vi "DiffDriveTrainSim_ClampInput.vi"(9 "BatteryVoltage":dbl, 11 "U":T1) -> (0 "Size Coerced":bool, 3 "Normalized U":T1)   [LabVIEW 2019, in "Trajectory_Library.lvlib"]
doc: "Clamp the input vector such that no element exceeds the battery voltage. If any does, the relative magnitudes of the input will be maintained.\n \nInputs:\n - u -- The input vector.\n - BatteryVoltage -- The battery voltage (volts)\n\nOutputs:\n - NormalizedU -- The normalized input.\n - SizeCoerced -- If TRUE, an error occured."
uses:
  Trajectory_Library.lvlib
  <vilib>/Analysis/Matrix/Datatypes/RealMatrix.ctl
  <vilib>/Analysis/Matrix/NI_Matrix.lvlib
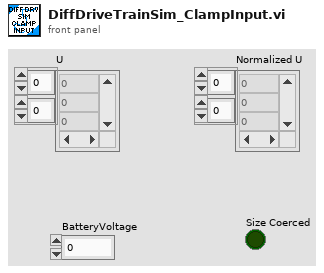
[diagram p1: front panel]
types:
  T1 = typedef "NI_Matrix.lvlib/RealMatrix.ctl" = dbl[][]
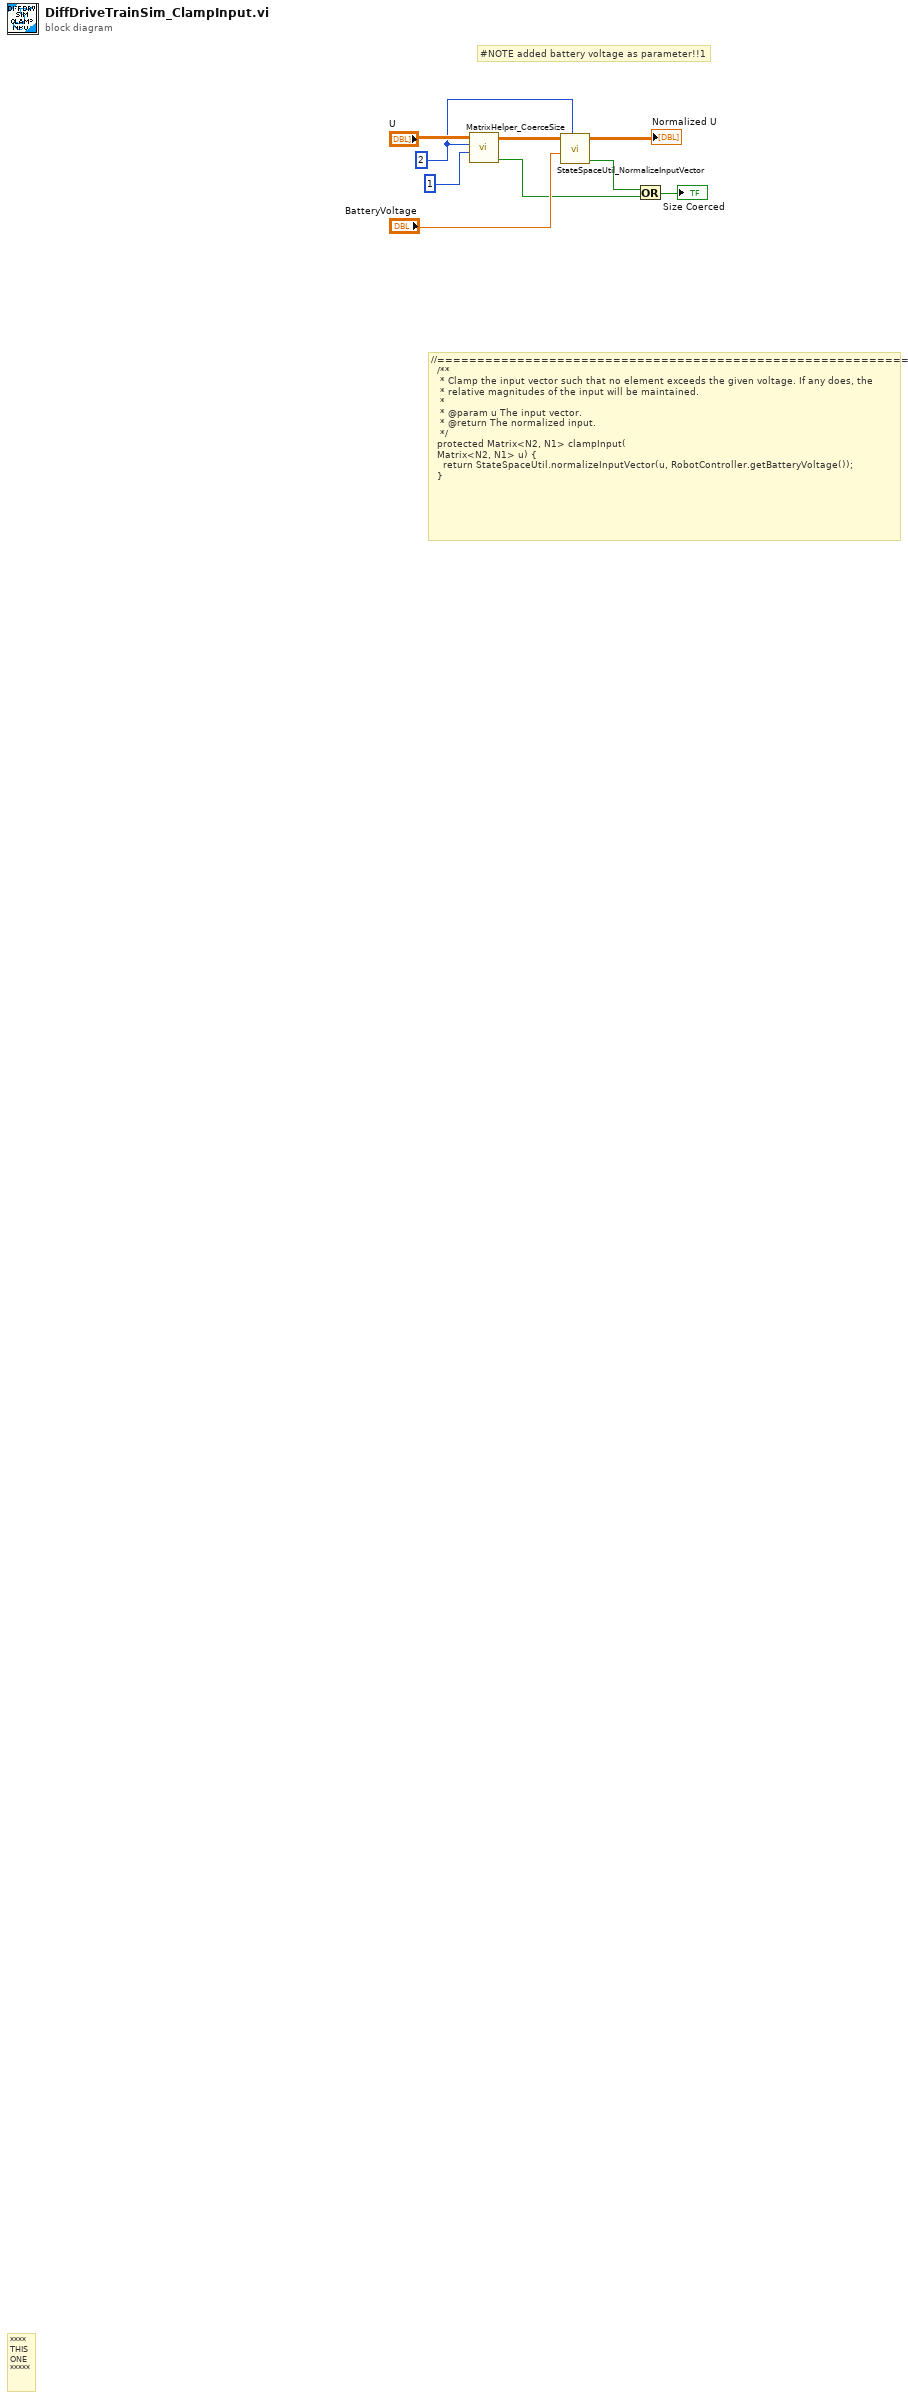
[diagram p0: block diagram]
diagram:
  w7 = 2 ("Rows")
  # "//============================================================\n  /**\n   * Clamp the input vector such that no element exceeds the given voltage. If any does, the\n   * relative magnitudes of the input will be maintained.\n   *\n   * @param u The input vector.\n   * @return The normalized input.\n   */\n  protected Matrix<N2, N1> clampInput(\n\t\tMatrix<N2, N1> u) {\n    return StateSpaceUtil.normalizeInputVector(u, RobotController.getBatteryVoltage());\n  }"
  # "#NOTE added battery voltage as parameter!!1"
  # "****\nTHIS\nONE\n*****"
  n1 = call "MatrixHelper_CoerceSize.vi"("Columns"=1, "Rows"=w7, "input matrix"="U") -> ("Coerced"=w2:bool, "output matrix"=w6:T1)  [unwired: 7 in]
  n2 = call "StateSpaceUtil_NormalizeInputVector.vi"("J"=w7, "Max_Magnitude"="BatteryVoltage", "U"=w6) -> ("Size Coerced"=w3:bool, "NormalizedU"=→"Normalized U":T1)  [unwired: 7 in]
  n3 = Or(x=w3, y=w2) -> (x .or. y?=→"Size Coerced":bool)
